vi "AddPAQtags.vi"(8 "error in (no error)":errorcluster, 9 "TAGs":string[](array[string]), 11 "AVPP in":refnum<class "AVPP.lvclass">) -> (0 "error out":errorcluster, 3 "AVPP out":refnum<class "AVPP.lvclass">)   [LabVIEW 2020, in "Sgraph_lib_V1.lvlib" / "AVPP.lvclass"]
doc: "This VI is usually called when new TAGs are sent using the HISW interface that do not yet exist.\nThis VI will check all TAG names of all Qtypes and if they do not exist: add them to PAQ tags.\nIf the supplied TAGs already exist in one of the other Qtypes: generate an error.\nTAG names must be unique whether they reside within its own or another Qtype area."
uses:
  AVPP.lvclass
  AVPP.lvclass/AVPP.ctl
  FAMM/FAMM.lvclass/FAMM.ctl
  Common/controls/typedef_com_TagProp.ctl
  DBAL/controls/DBAL_TAGpropEdit.ctl
  <vilib>/Utility/error.llb/Error Cluster From Error Code.vi
  <vilib>/ErrorRing/Error Ring.xnode
  DBAL/DBAL.lvclass
  FAMM/FAMM.lvclass
  Builds/Sgraph_lib_V1.lvlib
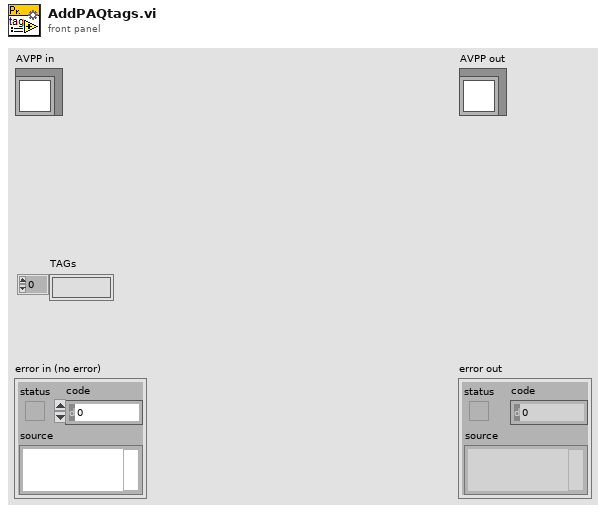
[diagram p1: front panel]
types:
  T1 = typedef "Sgraph_lib_V1.lvlib/DBAL_TAGpropEdit.ctl" = cluster{"TAG":string, "Qtype":string, "TAGprop":T2}
  T2 = typedef "Sgraph_lib_V1.lvlib/typedef_com_TagProp.ctl" = cluster{"Description":string, "EngUnits":string, "RangeH":dbl, "RangeL":dbl, "Resolution":i32, "Obsolete":bool, "ChangeDate":timestamp, "ChangeSource":string, "ChangeReason":string, "TagFunc":u32}
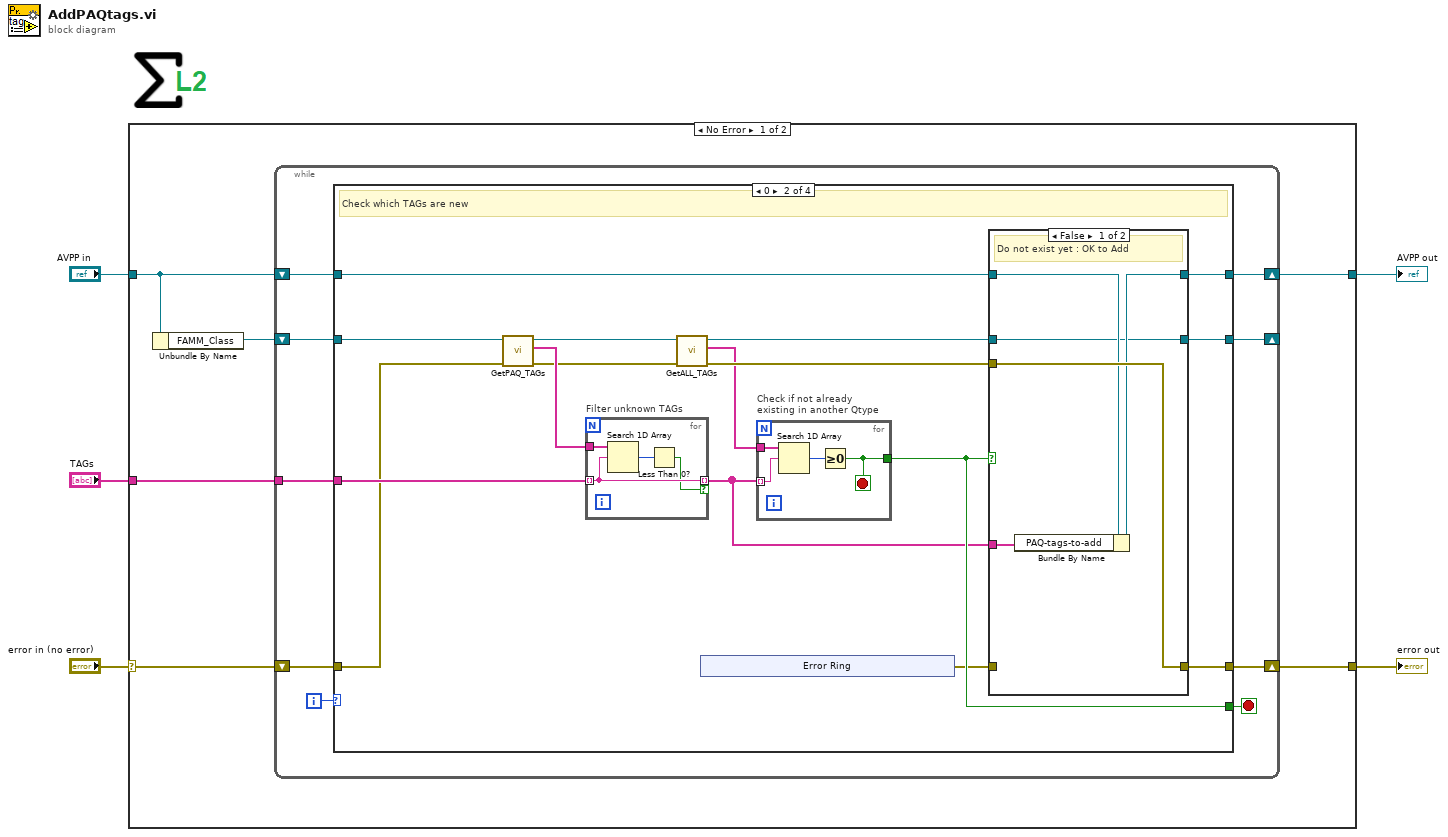
[diagram p0: block diagram]
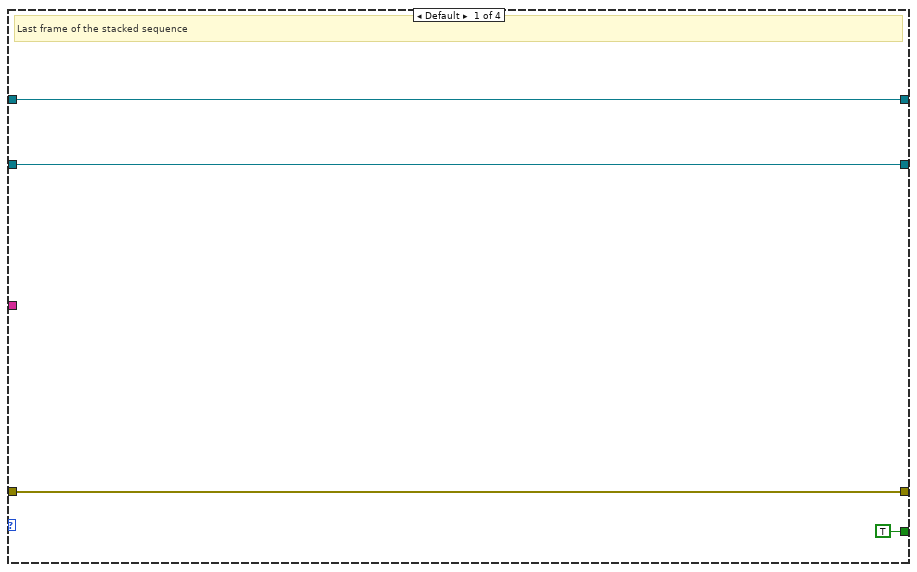
[diagram p2: hidden frame]
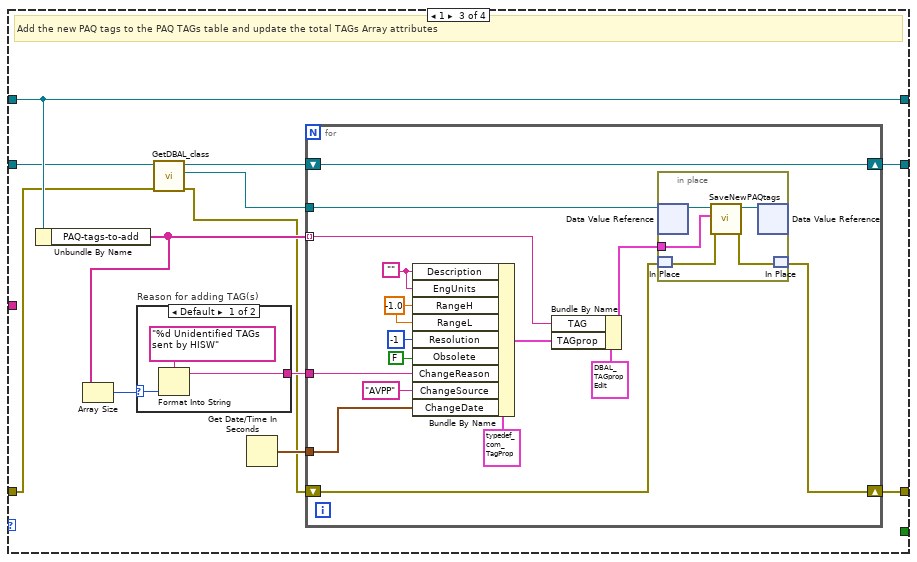
[diagram p4: hidden frame]
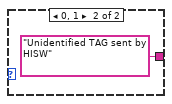
[diagram p5: hidden frame]
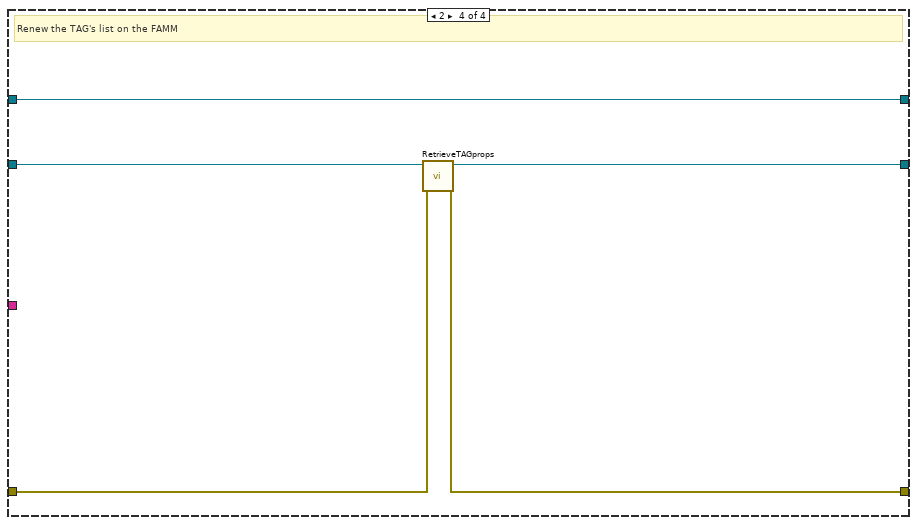
[diagram p6: hidden frame]
diagram:
  n1 = case shown="No Error" "error in (no error)" {
    selector: "error in (no error)" -> [w10 w105]
    tunnel: [w9 w105] -> w4
    tunnel: [w7 w104] -> w2
    tunnel: "AVPP in" -> [w8 w104]
    tunnel: "TAGs" -> [w11 _]
    frame No Error {
      n2 = Unbundle By Name(w8) -> ("FAMM_Class"=w6:refnum<class "FAMM.lvclass">)
      n3 = while {
        shift-right: [w18] -> _
        shift-left: w6 -> [w14]
        shift-right: [w16] -> w9
        shift-left: w10 -> [w17]
        tunnel: w11 -> [w15]
        shift-right: [w12] -> w7
        shift-left: w8 -> [w13]
        i -> [w20]
        stop <- w19 stop-if-true
        n4 = case shown="0" w20 {
          tunnel: [TRUE w38 _ _] -> w19
          tunnel: w14 -> [w23 w28 w66 w103]
          tunnel: [w23 w36 w72 w102] -> w18
          tunnel: w17 -> [w22 w39 w63 w101]
          tunnel: [w22 w34 w71 w100] -> w16
          tunnel: w15 -> [_ w40 _ _]
          tunnel: w13 -> [w21 w26 w67 w99]
          tunnel: [w21 w25 w67 w99] -> w12
          frame Default {
            # "Last frame of the stacked sequence"
          }
          frame 0 {
            # "Check which TAGs are new"
            n5 = call "GetPAQ_TAGs.vi"("error in (no error)"=w39, "FAMM in"=w28) -> ("error out"=w31:errorcluster, "PAQ_TAGs"=w32:string[], "FAMM out"=w30:refnum<class "FAMM.lvclass">)  [unwired: 7 in]
            n6 = for "Filter unknown TAGs" {
              tunnel: w32 -> [w48]
              tunnel: w40 -> [w46] mode=indexing
              tunnel: [w46] -> w35 mode=indexing if=w45
              n7 = Search 1D Array(1D array=w48, element=w46) -> (index of element=w47:i32)  [unwired: 1 in]
              n8 = Less Than 0?(x=w47) -> (x < 0?=w45:bool)
            }
            n9 = call "GetALL_TAGs.vi"("error in (no error)"=w31, "FAMM in"=w30) -> ("error out"=w37:errorcluster, "TAGs"=w29:string[], "FAMM out"=w27:refnum<class "FAMM.lvclass">)  [unwired: 7 in]
            n10 = xnode "Error Ring"() -> ("error out"=w33:errorcluster)
            n11 = for "Check if not already\nexisting in another Qtype" {
              tunnel: w29 -> [w44]
              tunnel: w35 -> [w42] mode=indexing
              tunnel: [w41] -> w38
              stop <- w41 stop-if-true
              n12 = Search 1D Array(1D array=w44, element=w42) -> (index of element=w43:i32)  [unwired: 1 in]
              n13 = Greater Or Equal To 0?(x=w43) -> (x >= 0?=w41:bool)
            }
            n14 = case shown="False" w38 {
              tunnel: w37 -> [w57 _]
              tunnel: w27 -> [w54 w61]
              tunnel: [w54 w61] -> w36
              tunnel: w35 -> [w58 _]
              tunnel: [w57 w60] -> w34
              tunnel: w33 -> [_ w60]
              tunnel: w26 -> [w56 w59]
              tunnel: [w55 w59] -> w25
              frame False {
                # "Do not exist yet : OK to Add"
                n15 = Bundle By Name(cluster=w56, "PAQ-tags-to-add"=w58) -> (w55:refnum<class "AVPP.lvclass">)
              }
              frame True {
                # "Duplicate TAG name !!"
              }
            }
          }
          frame 1 {
            # "Add the new PAQ tags to the PAQ TAGs table and update the total TAGs Array attributes"
            n16 = Unbundle By Name(w67) -> ("PAQ-tags-to-add"=w69:string[])
            n17 = Array Size(array=w69) -> (size(s)=w70:i32)
            n18 = case "Reason for adding TAG(s)" shown="Default" w70 {
              selector: w70 -> [w76 _]
              tunnel: [w74 "Unidentified TAG sent by HISW" ("ChangeSource")] -> w68
              frame Default {
                n19 = Format Into String(format string="%d Unidentified TAGs sent by HISW" ("ChangeSource"), w76) -> (resulting string=w74:string)  [unwired: 2 in, 1 out]
              }
              frame 0, 1 {
              }
            }
            n20 = call "GetDBAL_class.vi"("error in (no error)"=w63, "FAMM in"=w66) -> ("error out"=w62:errorcluster, "DBAL_class"=w64:refnum<data-value>, "FAMM out"=w65:refnum<class "FAMM.lvclass">)  [unwired: 7 in]
            n21 = Get Date/Time In Seconds() -> (seconds since 1Jan1904=w73:timestamp)
            n22 = for {
              tunnel: w69 -> [w85] mode=indexing
              shift-right: [w82] -> w72
              shift-left: w65 -> [w82]
              shift-right: [w83] -> w71
              shift-left: w62 -> [w80]
              tunnel: w73 -> [w79]
              tunnel: w64 -> [w81]
              tunnel: w68 -> [w78]
              w91 = -1.0 ("RangeH")
              w92 = ""
              n23 = Bundle By Name(cluster=T2 {"Description"="", "EngUnits"="", "RangeH"=0.0, "RangeL"=0.0, "Resolution"=0, "Obsolete"=FALSE, "ChangeDate"=timestamp(0 s since 1904-01-01), "ChangeSource"="", "ChangeReason"="", "TagFunc"=0} ("TAGprop"), "Description"=w92, "EngUnits"=w92, "RangeH"=w91, "RangeL"=w91, "Resolution"=-1, "Obsolete"=FALSE, "ChangeReason"=w78, "ChangeSource"="AVPP", "ChangeDate"=w79) -> (w86:T2)
              n24 = Bundle By Name(cluster=T1 {"TAG"="", "Qtype"="", "TAGprop"={"Description"="", "EngUnits"="", "RangeH"=0.0, "RangeL"=0.0, "Resolution"=0, "Obsolete"=FALSE, "ChangeDate"=timestamp(0 s since 1904-01-01), "ChangeSource"="", "ChangeReason"="", "TagFunc"=0}} ("TAGpropertyEdit"), "TAG"=w85, "TAGprop"=w86) -> (w84:T1)
              n25 = in-place {
                in-place-border: w84 -> [w94]
                n26 = in-place-dvr #1(w81) -> (w98:refnum<class "DBAL.lvclass">)  [unwired: 1 out]
                n27 = in-place-match #2(w80) -> (w97:errorcluster)
                n28 = call-dynamic "SaveNewPAQtags.vi"("error in (no error)"=w97, "TAGpropertyEdit"=w94, "DBAL in"=w98) -> ("error out"=w96:errorcluster, "DBAL out"=w95:refnum<class "DBAL.lvclass">)  [unwired: 7 in]
                n29 = in-place-dvr #1(w95) -> ()  [unwired: 2 out]
                n30 = in-place-match #2(w96) -> (w83:errorcluster)
              }
            }
          }
          frame 2 {
            # "Renew the TAG's list on the FAMM"
            n31 = call "RetrieveTAGprops.vi"("error in (no error)"=w101, "FAMM in"=w103) -> ("error out"=w100:errorcluster, "FAMM out"=w102:refnum<class "FAMM.lvclass">)  [unwired: 8 in]
          }
        }
      }
    }
    frame Error {
    }
  }
  "error out" <- w4
  "AVPP out" <- w2
